vi "Pre Launch Init.vi"(11 "ZM-CM-communication_manager in":refnum<class "ZM-CM-communication_manager.lvclass">) -> (0 "error out":errorcluster, 3 "ZM-CM-communication_manager out":refnum<class "ZM-CM-communication_manager.lvclass">)   [LabVIEW 2020, in "ZM-CM-communication_manager.lvlib" / "ZM-CM-communication_manager.lvclass"]
doc: "Pre Launch Init override of the communication manager: Call Parent, then ZM-CM-createResources initialises the protocol from the pre-launch settings. If that fails, what was opened is released and the error fails the launch (Stop Core does not run)."
uses:
  ZM-CM-communication_manager.lvclass
  <vilib>/ActorFramework/Actor/Actor.lvclass
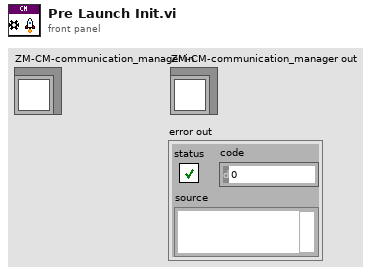
[diagram p1: front panel]
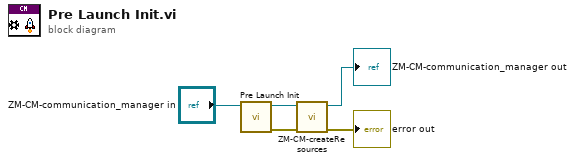
[diagram p0: block diagram]
diagram:
  n1 = call-parent "Pre Launch Init.vi"("Actor in"="ZM-CM-communication_manager in") -> ("error out"=w1:errorcluster, "Actor out"=w3:refnum<class "ZM-CM-communication_manager.lvclass">)  [unwired: 9 in]
  n2 = call "ZM-CM-createResources.vi"("error in (no error)"=w1, "ZM-CM-communication_manager in"=w3) -> ("error out"=→"error out":errorcluster, "ZM-CM-communication_manager out"=→"ZM-CM-communication_manager out":refnum<class "ZM-CM-communication_manager.lvclass">)  [unwired: 8 in]
